vi "Main.vi"() -> ()   [LabVIEW 2024]
doc: "Use this template to build a simple state machine design pattern. Each state executes code and determines which state to transition to."
uses:
  <vilib>/Analysis/Matrix/Datatypes/RealMatrix.ctl
  controls/State.ctl
  <vilib>/Platform/TimedLoop/XDataNode/timing_clust.ctl
  <vilib>/Platform/TimedLoop/XDataNode/nitl_modes.ctl
  <vilib>/Platform/TimedLoop/XDataNode/wakeup.ctl
  <vilib>/Analysis/Matrix/Numeric/Conversions/Array To Matrix - RA.vi
  <vilib>/platform/TimedLoop/XDataNode/XDataNode.xnode
  <vilib>/Platform/TimedLoop/XDataNode/XDNodeRunTimeDep.lvlib
  <vilib>/Analysis/Matrix/NI_Matrix.lvlib
panel:
  out "A Gate":dbl[](array[numeric])
  in  "N per point":i32=1
  in  "X and Y scale":T1(radio)
  out "Time left":dbl
  in  "Delay Time (s)":dbl=2.0
  out "Elapsed Time (s)":dbl
  out "Time has Elapsed":bool
  in  "y":dbl
  out "done with negative":bool=TRUE
  out "Y already happened":bool
  out "Is Y equal?":bool
  out "What am I scanning? T = X, F = Y":bool
  out "First go through?":bool
  out "X value":dbl
  in  "X":dbl(slide)=2.0852713584899902 scale=1.0..30.0 scale format="%#_2g"
  out "Y value":dbl
  in  "Y":dbl(slide)=2.050561797752809 scale=1.0..10.0 scale format="%#_3g"
  out "Numeric 2":dbl
  out "Numeric":dbl
  out "Come back X?":bool
  out "output array":dbl[][](array[numeric])
  out "Y graph":dbl
  out "X graph":dbl
  in  "element":dbl
  out "Y come back?":bool=TRUE
  out "Intensity Graph":dbl[][](graph)
  out "Distance traveled in mm X":dbl
  in  "Up":bool=TRUE
  out "Intensity Chart":dbl[][](graph)
  out "average values":T2
  out "x/y":dbl
  out "Distance traveled in mm Y":dbl
  out "element 2":dbl
  in  "Left":bool=TRUE
  in  "Step size mm  Y":dbl=0.005
  in  "Y Motor":refnum<k7>(container)
  in  "Step size mm X":dbl=0.005
  in  "X Motor":refnum<k7>(container)
  # "Distance to scan"
  # "Takes the nearest whole number\nAdjust before program starts"
  # "Movement"
  # "Right"
  # "Lowest Value for this motor is 0.008 mm"
  # "Down"
  # "Lowest value for this motor is 0.002 mm"
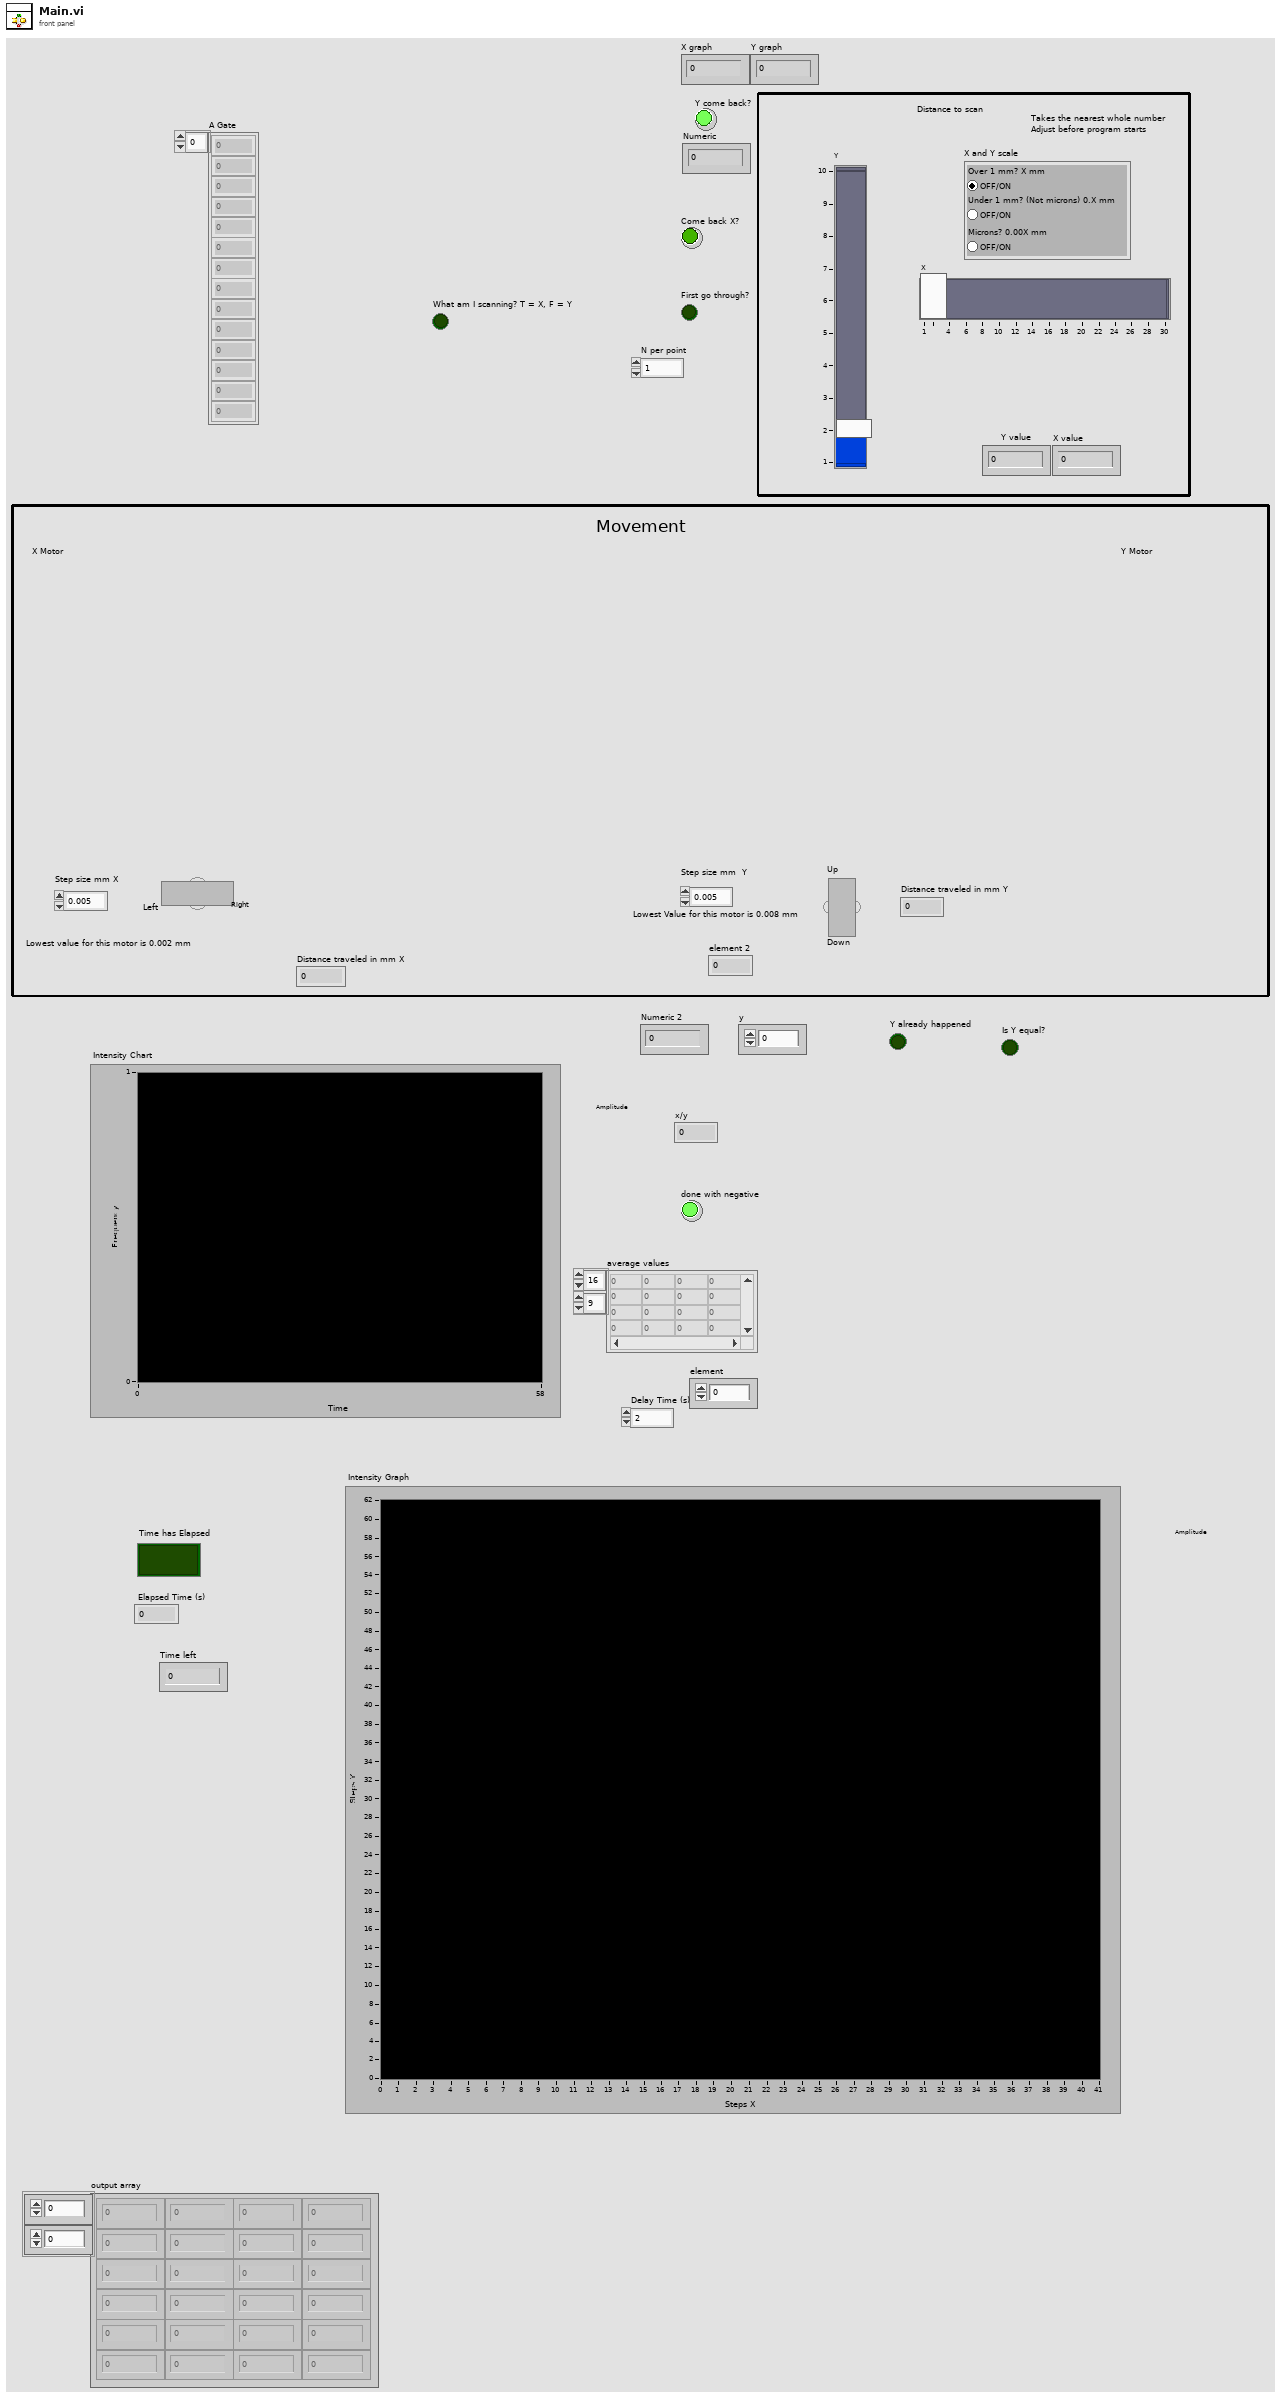
[diagram p1: front panel]
types:
  T1 = enum32{"Over 1 mm? X mm", "Under 1 mm? (Not microns) 0.X mm", "Microns? 0.00X mm"}
  T2 = typedef "NI_Matrix.lvlib/RealMatrix.ctl" = dbl[][]
  T3 = typedef "State.ctl" = enum16{"Initialize", "X Movement", "Y Movement", "Measurement", "Exit"}
  T4 = typedef "XDNodeRunTimeDep.lvlib/timing_clust.ctl" = cluster{"Expected End [f-1]":u64, "Actual End [f-1]":u64, "Finished Late? [f-1]":bool, "Expected End [i-1]":u64, "Actual End [i-1]":u64, "Finished Late? [i-1]":bool, "Expected Start [i]":u64, "Actual Start [i]":u64, "Expected Start [f]":u64, "Actual Start [f]":u64, "Source Name":string, "Structure Name":string, "Period":i64, "Deadline":i64, "Offset":i64, "Start":i64, "Priority":i32, "Timeout":i32, "Mode":T5, "Wakeup Reason":T6, "Error":errorcluster, "Source Type":string, "Secondary Source Type":string, "Global End Time":u64, "Global Start Time":u64, "Frame Duration":u64, "Iteration Duration":u64, "Assigned CPU":i32, "I/O Scan Engine Mode":u32}
  T5 = typedef "XDNodeRunTimeDep.lvlib/nitl_modes.ctl" = enum32{"No Change", "Process missed periods, maintain original phase", "Discard missed periods, maintain original phase", "Process missed periods, ignore original phase", "Discard missed periods, ignore original phase"}
  T6 = typedef "XDNodeRunTimeDep.lvlib/wakeup.ctl" = enum32{"Normal", "Aborted", "Asynchronous wakeup", "Timing source error", "Timed loop error", "Timeout"}
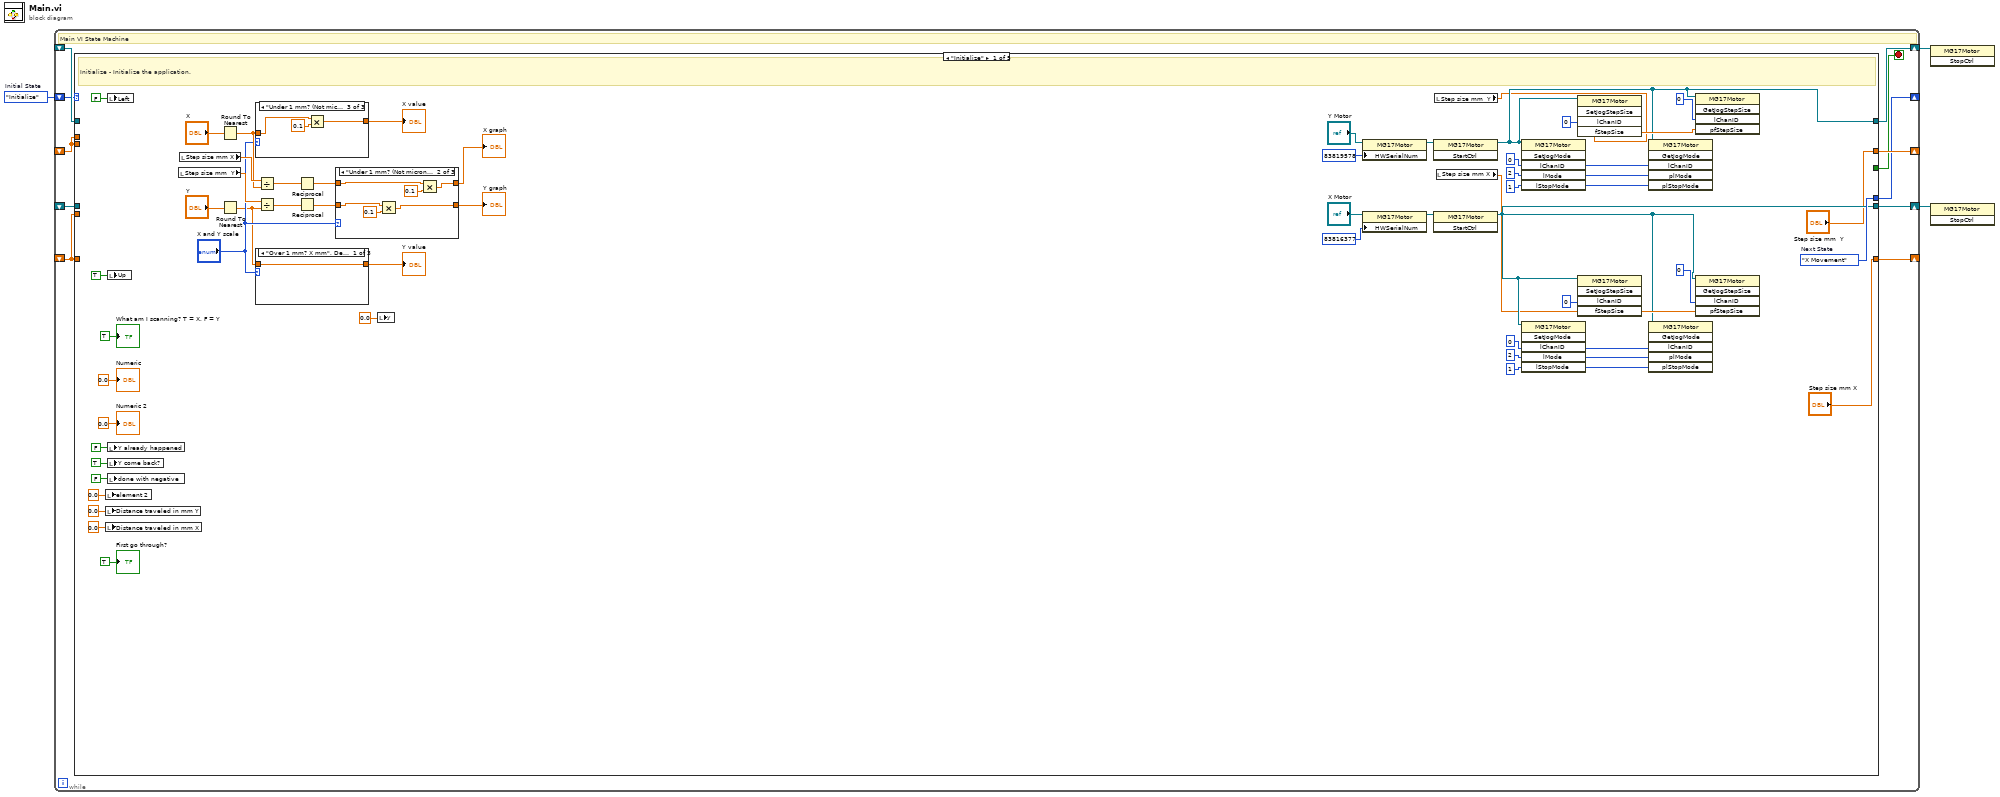
[diagram p0: block diagram]
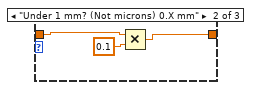
[diagram p2: hidden frame]
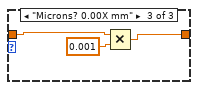
[diagram p3: hidden frame]
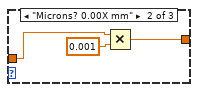
[diagram p5: hidden frame]
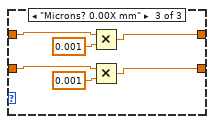
[diagram p7: hidden frame]
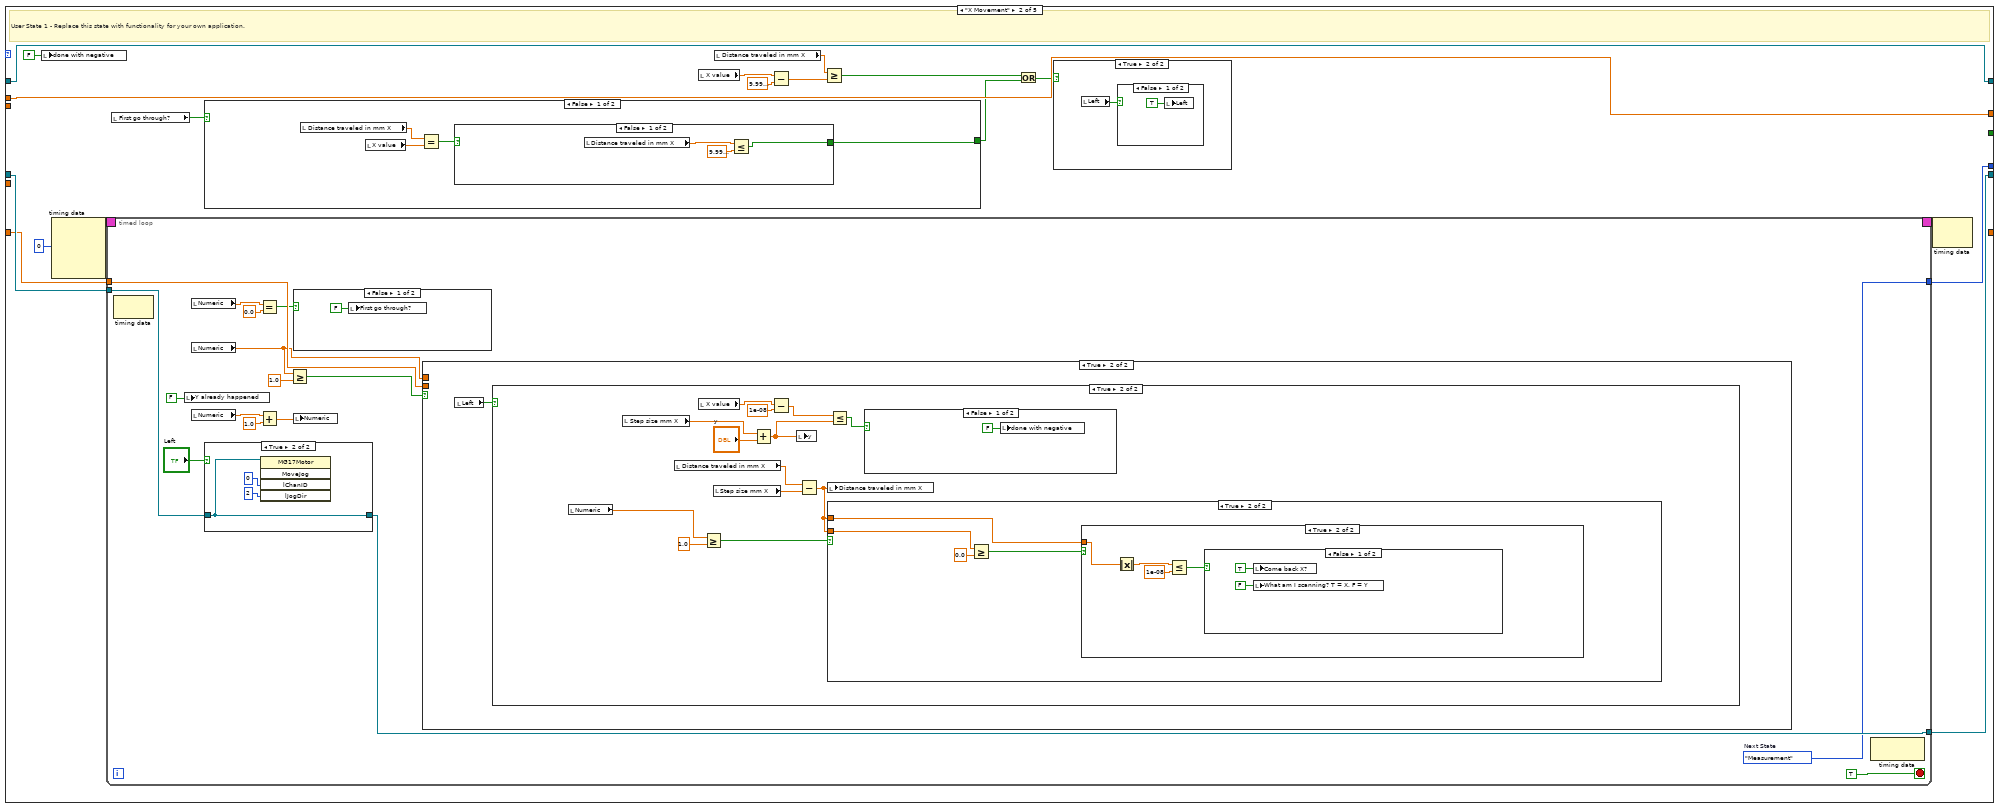
[diagram p8: hidden frame]
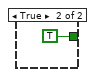
[diagram p9: hidden frame]
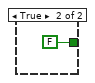
[diagram p10: hidden frame]
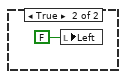
[diagram p12: hidden frame]
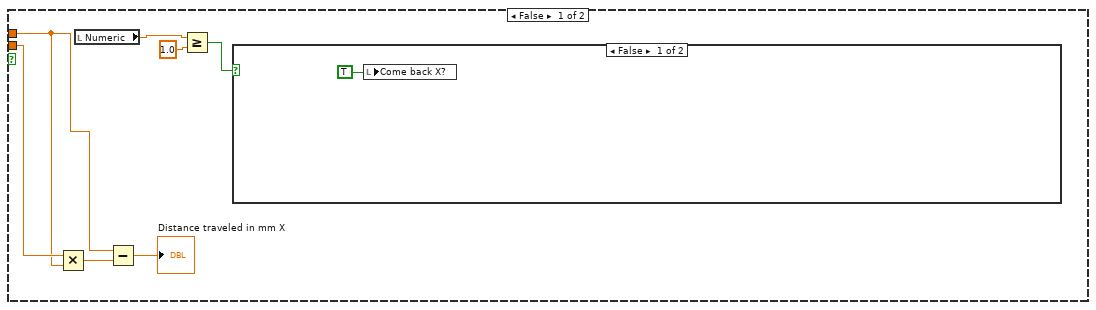
[diagram p14: hidden frame]
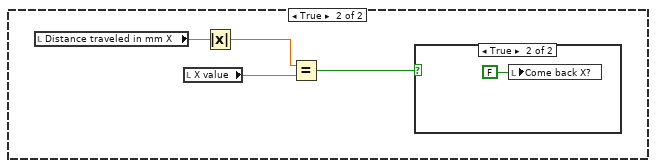
[diagram p15: hidden frame]
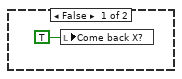
[diagram p16: hidden frame]
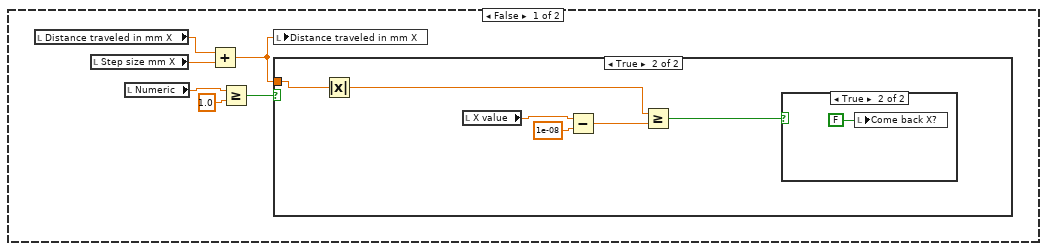
[diagram p17: hidden frame]
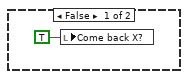
[diagram p18: hidden frame]
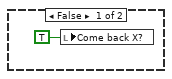
[diagram p19: hidden frame]
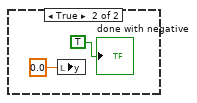
[diagram p20: hidden frame]
diagram:
  w3 = State."Initialize"  # Initial State
  n1 = while {
    shift-right: [w6] -> _
    shift-left: w3 -> [w7]
    shift-right: [w14] -> w2
    shift-left: _ -> [w12]
    shift-right: [w13] -> w1
    shift-left: _ -> [w9]
    shift-right: [w11] -> _
    shift-left: _ -> [w5]
    shift-right: [w10] -> _
    shift-left: _ -> [w4]
    stop <- w8 stop-if-true
    # "Main VI State Machine"
    n2 = case shown="\"Initialize\"" w7 {
      tunnel: [w73 w111 w223 w301 w338] -> w6
      tunnel: [w48 w118 w228 w295 w336] -> w14
      tunnel: [w47 w115 w230 w294 w337] -> w13
      tunnel: w12 -> [_ w119 w228 w295 w336]
      tunnel: ["Step size mm X" _ w227 _ w335] -> w11
      tunnel: ["Step size mm  Y" w116 _ _ w334] -> w10
      tunnel: w5 -> [_ w117 w227 _ w335]
      tunnel: w9 -> [_ w115 w231 w294 w337]
      tunnel: w4 -> [_ w116 w229 _ w334]
      tunnel: [_ _ _ _ w333] -> w8
      tunnel: w5 -> [_ _ _ _ _]
      tunnel: w4 -> [_ _ _ _ _]
      frame "Initialize" {
        w73 = State."X Movement"  # Next State
        # "Initialize - Initialize the application."
        n3 = local write "element 2"(0.0 ("element 2")) -> ()
        n4 = local write "Distance traveled in mm Y"(0.0 ("Distance traveled in mm Y")) -> ()
        n5 = local write "Distance traveled in mm X"(0.0 ("Distance traveled in mm X")) -> ()
        n6 = local write "Left"(FALSE) -> ()
        n7 = local write "Up"(TRUE ("Up")) -> ()
        n8 = local write "Y already happened"(FALSE ("Y already happened")) -> ()
        n9 = local write "Y come back?"(TRUE ("Y come back?")) -> ()
        n10 = local write "done with negative"(FALSE) -> ()
        n11 = local read "Step size mm  Y"() -> (w42:dbl)
        n12 = local read "Step size mm X"() -> (w37:dbl)
        n13 = Round To Nearest(number="X") -> (nearest integer value=w19:dbl)
        n14 = Round To Nearest(number="Y") -> (nearest integer value=w16:dbl)
        n15 = case shown="\"Under 1 mm? (Not microns) 0.X mm\"" "X and Y scale" {
          tunnel: w19 -> [w81 w84 w87]
          tunnel: [w81 w82 w85] -> w18
          frame "Over 1 mm? X mm", Default {
          }
          frame "Microns? 0.00X mm" {
            n16 = Multiply(x=w84, y=0.001) -> (x*y=w82:dbl)
          }
          frame "Under 1 mm? (Not microns) 0.X mm" {
            n17 = Multiply(x=w87, y=0.1) -> (x*y=w85:dbl)
          }
        }
        "X value" <- w18
        n18 = case shown="\"Over 1 mm? X mm\", Default" "X and Y scale" {
          tunnel: w16 -> [w74 w75 w80]
          tunnel: [w74 w76 w78] -> w15
          frame "Over 1 mm? X mm", Default {
          }
          frame "Under 1 mm? (Not microns) 0.X mm" {
            n19 = Multiply(x=w75, y=0.1) -> (x*y=w76:dbl)
          }
          frame "Microns? 0.00X mm" {
            n20 = Multiply(x=w80, y=0.001) -> (x*y=w78:dbl)
          }
        }
        "Y value" <- w15
        n21 = Divide(x=w37, y=w19) -> (x/y=w38:dbl)
        n22 = Divide(x=w42, y=w16) -> (x/y=w41:dbl)
        n23 = Reciprocal(x=w38) -> (1/x=w23:dbl)
        n24 = Reciprocal(x=w41) -> (1/x=w22:dbl)
        n25 = case shown="\"Under 1 mm? (Not microns) 0.X mm\"" "X and Y scale" {
          tunnel: w23 -> [w88 w95 w101]
          tunnel: w22 -> [w89 w92 w98]
          tunnel: [w88 w93 w99] -> w21
          tunnel: [w89 w90 w96] -> w20
          frame "Over 1 mm? X mm", Default {
          }
          frame "Under 1 mm? (Not microns) 0.X mm" {
            n26 = Multiply(x=w92, y=0.1) -> (x*y=w90:dbl)
            n27 = Multiply(x=w95, y=0.1) -> (x*y=w93:dbl)
          }
          frame "Microns? 0.00X mm" {
            n28 = Multiply(x=w101, y=0.001) -> (x*y=w99:dbl)
            n29 = Multiply(x=w98, y=0.001) -> (x*y=w96:dbl)
          }
        }
        "Y graph" <- w20
        "X graph" <- w21
        n30 = local write "y"(0.0 ("y")) -> ()
        n31 = property class="MG17Motor"(reference="Y Motor", "HWSerialNum"=83819578) -> (reference out=w58:refnum<k7>)  [unwired: 1 in, 1 out]
        n32 = property class="MG17Motor"(reference="X Motor", "HWSerialNum"=83816377) -> (reference out=w70:refnum<k7>)  [unwired: 1 in, 1 out]
        n33 = invoke class="MG17Motor" method="StartCtrl"(reference=w58) -> (reference out=w47:refnum<k7>)  [unwired: 2 in, 2 out]
        n34 = invoke class="MG17Motor" method="StartCtrl"(reference=w70) -> (reference out=w48:refnum<k7>)  [unwired: 2 in, 2 out]
        n35 = local read "Step size mm  Y"() -> (w24:dbl)
        n36 = local read "Step size mm X"() -> (w25:dbl)
        n37 = invoke class="MG17Motor" method="SetJogMode"(reference=w47, "lChanID"=0, "lMode"=2, "lStopMode"=1) -> ("lChanID"=w49:i32, "lMode"=w50:i32, "lStopMode"=w51:i32)  [unwired: 2 in, 3 out]
        n38 = invoke class="MG17Motor" method="SetJogMode"(reference=w48, "lChanID"=0, "lMode"=2, "lStopMode"=1) -> ("lChanID"=w61:i32, "lMode"=w62:i32, "lStopMode"=w63:i32)  [unwired: 2 in, 3 out]
        n39 = invoke class="MG17Motor" method="SetJogStepSize"(reference=w47, "lChanID"=0, "fStepSize"=w24) -> ("fStepSize"=w55:sgl)  [unwired: 2 in, 4 out]
        n40 = invoke class="MG17Motor" method="SetJogStepSize"(reference=w48, "lChanID"=0, "fStepSize"=w25) -> ("fStepSize"=w67:sgl)  [unwired: 2 in, 4 out]
        n41 = invoke class="MG17Motor" method="GetJogMode"(reference=w47, "lChanID"=w49, "plMode"=w50, "plStopMode"=w51) -> ()  [unwired: 2 in, 6 out]
        n42 = invoke class="MG17Motor" method="GetJogMode"(reference=w48, "lChanID"=w61, "plMode"=w62, "plStopMode"=w63) -> ()  [unwired: 2 in, 6 out]
        n43 = invoke class="MG17Motor" method="GetJogStepSize"(reference=w47, "lChanID"=0, "pfStepSize"=w55) -> ()  [unwired: 2 in, 5 out]
        n44 = invoke class="MG17Motor" method="GetJogStepSize"(reference=w48, "lChanID"=0, "pfStepSize"=w67) -> ()  [unwired: 2 in, 5 out]
        "Numeric" <- 0.0
        "Numeric 2" <- 0.0
        "First go through?" <- TRUE
        "What am I scanning? T = X, F = Y" <- TRUE
      }
      frame "X Movement" {
        # "User State 1 - Replace this state with functionality for your own application."
        n45 = local write "done with negative"(FALSE) -> ()
        n46 = node-c288(i64 0 ("Period")) -> (w114:T4)  [unwired: 3 in]
        n47 = timed-loop {
          tunnel: [w146] -> w118
          tunnel: w119 -> [w147]
          timing: w114 -> [_]
          timing-out: [_] -> w113
          tunnel: w117 -> [w143]
          tunnel: [w140] -> w111
          stop <- TRUE stop-if-true
          w140 = State."Measurement"  # Next State
          n48 = node-c288() -> ()  [unwired: 1 in, 1 out]
          n49 = local write "Y already happened"(FALSE ("Y already happened")) -> ()
          n50 = local read "Numeric"() -> (w136:dbl)
          n51 = local read "Numeric"() -> (w132:dbl)
          n52 = local read "Numeric"() -> (w137:dbl)
          n53 = case shown="True" "Left" {
            tunnel: w147 -> [w213 w216]
            tunnel: [w213 w216] -> w146
            frame False {
              n54 = invoke class="MG17Motor" method="MoveJog"(reference=w213, "lChanID"=0, "lJogDir"=1) -> ()  [unwired: 2 in, 5 out]
            }
            frame True {
              n55 = invoke class="MG17Motor" method="MoveJog"(reference=w216, "lChanID"=0, "lJogDir"=2) -> ()  [unwired: 2 in, 5 out]
            }
          }
          n56 = Equal?(x=w136, y=0.0) -> (x = y?=w134:bool)
          n57 = Add(x=w137, y=1.0) -> (x+y=w138:dbl)
          n58 = Greater Or Equal?(x=w132, y=1.0) -> (x >= y?=w144:bool)
          n59 = case shown="False" w134 {
            frame False {
              n60 = local write "First go through?"(FALSE ("First go through?")) -> ()
            }
            frame True {
            }
          }
          n61 = local write "Numeric"(w138) -> ()
          n62 = case shown="True" w144 {
            tunnel: w143 -> [w154 _]
            tunnel: w132 -> [w153 _]
            frame False {
              n63 = Multiply(x=w154, y=w153) -> (x*y=w155:dbl)
              n64 = local read "Numeric"() -> (w152:dbl)
              n65 = Subtract(x=w153, y=w155) -> (x-y=→"Distance traveled in mm X":dbl)
              n66 = Greater Or Equal?(x=w152, y=1.0) -> (x >= y?=w150:bool)
              n67 = case shown="False" w150 {
                frame False {
                  n68 = local write "Come back X?"(TRUE ("Come back X?")) -> ()
                }
                frame True {
                  n69 = local read "Distance traveled in mm X"() -> (w160:dbl)
                  n70 = local read "X value"() -> (w158:dbl)
                  n71 = Absolute Value(x=w160) -> (abs(x)=w159:dbl)
                  n72 = Equal?(x=w159, y=w158) -> (x = y?=w157:bool)
                  n73 = case shown="True" w157 {
                    frame False {
                      n74 = local write "Come back X?"(TRUE ("Come back X?")) -> ()
                    }
                    frame True {
                      n75 = local write "Come back X?"(FALSE ("Come back X?")) -> ()
                    }
                  }
                }
              }
            }
            frame True {
              n76 = local read "Left"() -> (w163:bool)
              n77 = case shown="True" w163 {
                frame False {
                  n78 = local read "Distance traveled in mm X"() -> (w169:dbl)
                  n79 = local read "Step size mm X"() -> (w168:dbl)
                  n80 = local read "Numeric"() -> (w166:dbl)
                  n81 = Add(x=w169, y=w168) -> (x+y=w164:dbl)
                  n82 = Greater Or Equal?(x=w166, y=1.0) -> (x >= y?=w165:bool)
                  n83 = local write "Distance traveled in mm X"(w164) -> ()
                  n84 = case shown="True" w165 {
                    tunnel: w164 -> [_ w174]
                    frame False {
                      n85 = local write "Come back X?"(TRUE ("Come back X?")) -> ()
                    }
                    frame True {
                      n86 = Absolute Value(x=w174) -> (abs(x)=w176:dbl)
                      n87 = local read "X value"() -> (w173:dbl)
                      n88 = Subtract(x=w173, y=1e-08) -> (x-y=w171:dbl)
                      n89 = Greater Or Equal?(x=w176, y=w171) -> (x >= y?=w175:bool)
                      n90 = case shown="True" w175 {
                        frame False {
                          n91 = local write "Come back X?"(TRUE ("Come back X?")) -> ()
                        }
                        frame True {
                          n92 = local write "Come back X?"(FALSE ("Come back X?")) -> ()
                        }
                      }
                    }
                  }
                }
                frame True {
                  n93 = local read "Numeric"() -> (w188:dbl)
                  n94 = local read "Step size mm X"() -> (w185:dbl)
                  n95 = local read "Distance traveled in mm X"() -> (w191:dbl)
                  n96 = local read "X value"() -> (w182:dbl)
                  n97 = Greater Or Equal?(x=w188, y=1.0) -> (x >= y?=w187:bool)
                  n98 = local read "Step size mm X"() -> (w190:dbl)
                  n99 = Add(x=w185, y="y") -> (x+y=w183:dbl)
                  n100 = Subtract(x=w182, y=1e-08) -> (x-y=w180:dbl)
                  n101 = local write "y"(w183) -> ()
                  n102 = Subtract(x=w191, y=w190) -> (x-y=w179:dbl)
                  n103 = local write "Distance traveled in mm X"(w179) -> ()
                  n104 = case shown="True" w187 {
                    tunnel: w179 -> [_ w197]
                    tunnel: w179 -> [_ w198]
                    frame False {
                      n105 = local write "Come back X?"(TRUE) -> ()
                    }
                    frame True {
                      n106 = Greater Or Equal?(x=w198, y=0.0) -> (x >= y?=w199:bool)
                      n107 = case shown="True" w199 {
                        tunnel: w197 -> [_ w204]
                        frame False {
                          n108 = local read "Is Y equal?"() -> (w200:bool)
                          n109 = case shown="False" w200 {
                            frame False {
                              n110 = local write "Come back X?"(TRUE) -> ()
                            }
                            frame True {
                              n111 = local write "Come back X?"(FALSE ("Come back X?")) -> ()
                            }
                          }
                        }
                        frame True {
                          n112 = Absolute Value(x=w204) -> (abs(x)=w206:dbl)
                          n113 = Less Or Equal?(x=w206, y=1e-08) -> (x <= y?=w205:bool)
                          n114 = case shown="False" w205 {
                            frame False {
                              n115 = local write "Come back X?"(TRUE) -> ()
                              n116 = local write "What am I scanning? T = X, F = Y"(FALSE) -> ()
                            }
                            frame True {
                              n117 = local write "What am I scanning? T = X, F = Y"(TRUE) -> ()
                              "Come back X?" <- FALSE
                            }
                          }
                        }
                      }
                    }
                  }
                  n118 = Less Or Equal?(x=w180, y=w183) -> (x <= y?=w186:bool)
                  n119 = case shown="False" w186 {
                    frame False {
                      n120 = local write "done with negative"(FALSE) -> ()
                    }
                    frame True {
                      n121 = local write "y"(sgl 0.0 ("y")) -> ()
                      "done with negative" <- TRUE
                    }
                  }
                }
              }
            }
          }
          n122 = node-c288() -> ()  [unwired: 1 in, 1 out]
        }
        n123 = local read "First go through?"() -> (w109:bool)
        n124 = case shown="False" w109 {
          tunnel: [w120 FALSE] -> w108
          frame False {
            n125 = local read "Distance traveled in mm X"() -> (w123:dbl)
            n126 = local read "X value"() -> (w122:dbl)
            n127 = Equal?(x=w123, y=w122) -> (x = y?=w121:bool)
            n128 = case shown="False" w121 {
              tunnel: [w124 TRUE] -> w120
              frame False {
                n129 = local read "Distance traveled in mm X"() -> (w126:dbl)
                n130 = Less Or Equal?(x=w126, y=9.99999993922529e-09) -> (x <= y?=w124:bool)
              }
              frame True {
              }
            }
          }
          frame True {
          }
        }
        n131 = local read "X value"() -> (w106:dbl)
        n132 = local read "Distance traveled in mm X"() -> (w103:dbl)
        n133 = Subtract(x=w106, y=9.99999993922529e-09) -> (x-y=w104:dbl)
        n134 = Greater Or Equal?(x=w103, y=w104) -> (x >= y?=w107:bool)
        n135 = Or(x=w107, y=w108) -> (x .or. y?=w110:bool)
        n136 = case shown="True" w110 {
          frame False {
          }
          frame True {
            n137 = local read "Left"() -> (w129:bool)
            n138 = case shown="False" w129 {
              frame False {
                n139 = local write "Left"(TRUE) -> ()
              }
              frame True {
                n140 = local write "Left"(FALSE) -> ()
              }
            }
          }
        }
        n141 = node-c288(w113) -> ()  [unwired: 1 out]
      }
      frame "Y Movement" {
        w223 = State."Measurement"  # Next State
        # "User State 2 - Replace this state with functionality for your own application."
        n142 = node-c288(i64 0 ("Period")) -> (w226:T4)  [unwired: 3 in]
        n143 = timed-loop {
          timing: w226 -> [_]
          timing-out: [_] -> w225
          tunnel: w229 -> [w258]
          tunnel: w231 -> [w260]
          tunnel: [w259] -> w230
          stop <- w245 stop-if-true
          n144 = node-c288() -> ()  [unwired: 1 in, 1 out]
          n145 = local read "Numeric 2"() -> (w240:dbl)
          n146 = case shown="True" "Up" {
            tunnel: w260 -> [w263 w266]
            tunnel: [w263 w266] -> w259
            frame False {
              n147 = invoke class="MG17Motor" method="MoveJog"(reference=w263, "lChanID"=0, "lJogDir"=1) -> ()  [unwired: 2 in, 5 out]
            }
            frame True {
              n148 = invoke class="MG17Motor" method="MoveJog"(reference=w266, "lChanID"=0, "lJogDir"=2) -> ()  [unwired: 2 in, 5 out]
            }
          }
          n149 = local read "Step size mm  Y"() -> (w235:dbl)
          n150 = local read "Distance traveled in mm Y"() -> (w243:dbl)
          n151 = Add(x=w240, y=1.0) -> (x+y=w232:dbl)
          n152 = Multiply(x=w258, y=w232) -> (x*y=w257:dbl)
          n153 = Divide(x=w232, y=w235) -> (x/y=w234:dbl)
          n154 = local write "Numeric 2"(w232) -> ()
          n155 = Reciprocal(x=w234) -> (1/x=w233:dbl)
          n156 = Subtract(x=w232, y=w257) -> (x-y=w242:dbl)
          n157 = local read "Y value"() -> (w236:dbl)
          n158 = Add(x=w243, y=w242) -> (x+y=→"Distance traveled in mm Y":dbl)
          n159 = Initialize Array(w242, 100 ("dimension size")) -> (w255:dbl[])
          n160 = Greater Or Equal?(x=w233, y=w236) -> (x >= y?=w237:bool)
          "Is Y equal?" <- w237
          n161 = call-poly <vilib>:"Array To Matrix.vi"("Real 1D Array"=w255) -> ("Real Matrix (Column Vector)"=w254:T2)
          n162 = Replace Array Subset(array=w254, new element=w242, index (row)=0, index (col)=0) -> (w251:T2)
          n163 = case shown="False" w237 {
            frame False {
              n164 = local write "Y come back?"(TRUE) -> ()
            }
            frame True {
              "Y come back?" <- FALSE
            }
          }
          n165 = Index Array(array=w251, index (row)=0, index (col)=0) -> (element=→"element 2":dbl)
          n166 = Greater Or Equal?(x=0, y=0) -> (x >= y?=w245:bool)
          n167 = node-c288() -> ()  [unwired: 1 in, 1 out]
          "Y already happened" <- TRUE ("Y already happened")
        }
        n168 = node-c288(w225) -> ()  [unwired: 1 out]
      }
      frame "Measurement" {
        n169 = call "GPIB_SR400_A.vi"("N per point"="N per point") -> ("A Gate"=→"A Gate":dbl[], "x/y"=w277:dbl)  [unwired: 9 in]
        n170 = call "Time Delay2"("Delay Time (s)"="Delay Time (s)") -> ()  [unwired: 10 in, 1 out]
        n171 = Reciprocal(x=w277) -> (1/x=w293:dbl)
        "x/y" <- w293
        n172 = local read "First go through?"() -> (w300:bool)
        n173 = Build Array(w293) -> (w298:T2)
        "average values" <- w298
        "Intensity Chart" <- w298
        n174 = case shown="False" w300 {
          tunnel: w298 -> [_ w332]
          tunnel: [w324 w329] -> w299
          frame False {
            n175 = local read "output array"() -> (w324:dbl[][])
          }
          frame True {
            n176 = local read "Y graph"() -> (w326:dbl)
            n177 = local read "X graph"() -> (w327:dbl)
            n178 = Increment(x=w326) -> (x+1=w325:dbl)
            n179 = local read "Distance traveled in mm X"() -> (w330:dbl)
            n180 = Initialize Array("element", w327, w325) -> (w328:dbl[][])
            n181 = Insert Into Array(array=w328, index (row)=w330, new element=w332) -> (w329:dbl[][])  [unwired: 1 in]
          }
        }
        n182 = local read "X graph"() -> (w290:dbl)
        n183 = local read "Y graph"() -> (w289:dbl)
        n184 = local read "Delay Time (s)"() -> (w282:dbl)
        n185 = Multiply(x=w290, y=w289) -> (x*y=w288:dbl)
        n186 = Multiply(x=w288, y=w282) -> (x*y=w287:dbl)
        n187 = Add(x=w287, y=30.0) -> (x+y=w281:dbl)
        n188 = call "Elapsed Time"("Time Target (s)"=w281) -> ("Elapsed Time (s)"=w280:dbl, "Time has Elapsed"=w284:bool)  [unwired: 11 in, 6 out]
        "Time has Elapsed" <- w284
        "Elapsed Time (s)" <- w280
        n189 = local read "Distance traveled in mm X"() -> (w291:dbl)
        n190 = local read "Step size mm X"() -> (w292:dbl)
        n191 = Subtract(x=w281, y=w280) -> (x-y=→"Time left":dbl)
        n192 = Not(x=w284) -> (.not. x?=w285:bool)
        n193 = local read "Numeric 2"() -> (w296:dbl)
        n194 = case shown="True" w285 {
          tunnel: [w302 w306] -> w301
          frame False {
            w302 = State."Exit"  # Next State
          }
          frame True {
            n195 = local read "Come back X?"() -> (w308:bool)
            n196 = local read "Y come back?"() -> (w307:bool)
            n197 = local read "Is Y equal?"() -> (w303:bool)
            n198 = Or(x=w308, y=w307) -> (x .or. y?=w305:bool)
            n199 = Or(x=w303, y=w305) -> (x .or. y?=w304:bool)
            n200 = case shown="True" w304 {
              tunnel: [w309 w310] -> w306
              frame False {
                w309 = State."Exit"  # Next State
              }
              frame True {
                n201 = local read "Come back X?"() -> (w311:bool)
                n202 = case shown="True" w311 {
                  tunnel: [w312 w318] -> w310
                  frame False {
                    n203 = local read "Y already happened"() -> (w313:bool)
                    n204 = case shown="True" w313 {
                      tunnel: [w316 w317] -> w312
                      frame False {
                        w316 = State."Y Movement"  # Next State
                        n205 = local write "y"(0.0 ("y")) -> ()
                        n206 = local write "Y already happened"(FALSE ("Y already happened")) -> ()
                      }
                      frame True {
                        w317 = State."X Movement"  # Next State
                      }
                    }
                  }
                  frame True {
                    n207 = local read "done with negative"() -> (w319:bool)
                    n208 = case shown="False" w319 {
                      tunnel: [w320 w323] -> w318
                      frame False {
                        w320 = State."X Movement"  # Next State
                      }
                      frame True {
                        w323 = State."Y Movement"  # Next State
                        n209 = local write "y"(sgl 0.0 ("y")) -> ()
                        n210 = local write "done with negative"(FALSE) -> ()
                      }
                    }
                  }
                }
              }
            }
          }
        }
        n211 = Divide(x=w291, y=w292) -> (x/y=w297:dbl)
        n212 = Replace Array Subset "Replace Array Subset"(array=w299, new element=w293, index (row)=w297, index (col)=w296) -> (→"Intensity Graph" →"output array":dbl[][])
      }
      frame "Exit" {
        w333 = TRUE  # Stop Loop?
        w338 = State."Exit"  # (Value Not Used)
        # "The state value is not used here since this is the last iteration of the state machine loop."
        # "Exit - Exit the application."
      }
    }
  }
  n213 = invoke class="MG17Motor" method="StopCtrl"(reference=w1) -> ()  [unwired: 2 in, 3 out]
  n214 = invoke class="MG17Motor" method="StopCtrl"(reference=w2) -> ()  [unwired: 2 in, 3 out]
